vi "Close.vi"(8 "error in":errorcluster, 11 "Server in":refnum<class "Server.lvclass">) -> (0 "error out":errorcluster)   [LabVIEW 2020, in "PV Access.lvlib" / "PVA Server.lvlib" / "Server.lvclass"]
doc: "Close the server."
uses:
  Server.lvclass
  PV Access.lvlib
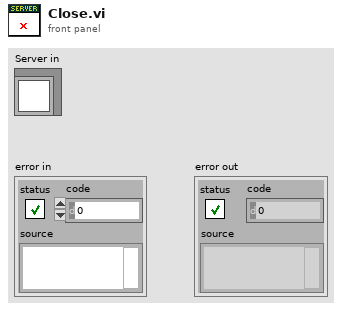
[diagram p1: front panel]
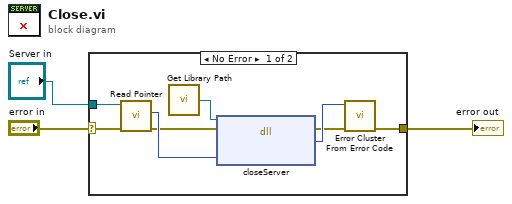
[diagram p0: block diagram]
diagram:
  n1 = case shown="No Error" "error in" {
    selector: "error in" -> [w4 w12]
    tunnel: [w11 w12] -> w3
    tunnel: "Server in" -> [w5 _]
    frame No Error {
      n2 = call-dynamic "Read Pointer.vi"("error in (no error)"=w4, "Pointer Base in"=w5) -> ("error out"=w6:errorcluster, "Pointer"=w7:i64)  [unwired: 7 in, 1 out]
      n3 = call "Get Library Path.vi"() -> ("Path"=w8:path)  [unwired: 1 in]
      n4 = dll-call lib="?" fn="closeServer"(path in=w8, error in=w6, "server"=w7) -> (error out=w9:errorcluster, "ret code"=w10:i32)  [unwired: 2 in, 1 out]
      n5 = call <vilib>:"Error Cluster From Error Code.vi"("error in (no error)"=w9, "error code (0)"=w10) -> ("error out"=w11:errorcluster)  [unwired: 7 in]
    }
    frame Error {
    }
  }
  "error out" <- w3
